vi "CD Storage Library Load.vi"(8 "error in (no error)":errorcluster, 11 "DMA Channel Testing in":refnum<class "FPGA Addon DMA Channel Unit Tests.lvclass">) -> (0 "error out":errorcluster, 3 "DMA Channel Testing out":refnum<class "FPGA Addon DMA Channel Unit Tests.lvclass">)   [LabVIEW 2020, in "FPGA Addon DMA Channel Unit Tests.lvclass"]
uses:
  FPGA Addon DMA Channel Unit Tests.lvclass
  FPGA Addon DMA Channel Unit Tests.lvclass/FPGA Addon DMA Channel Unit Tests.ctl
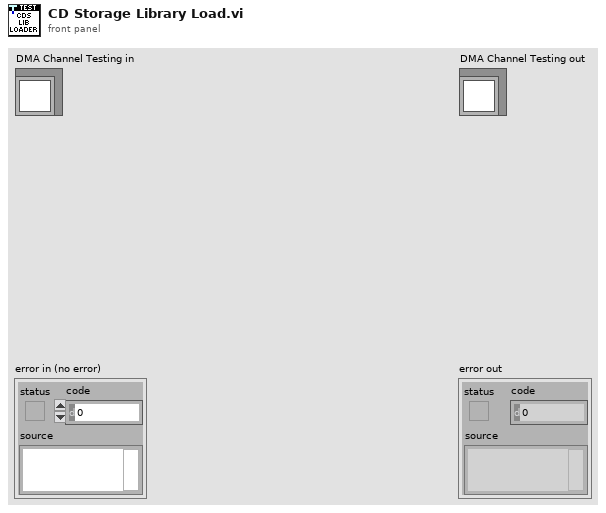
[diagram p1: front panel]
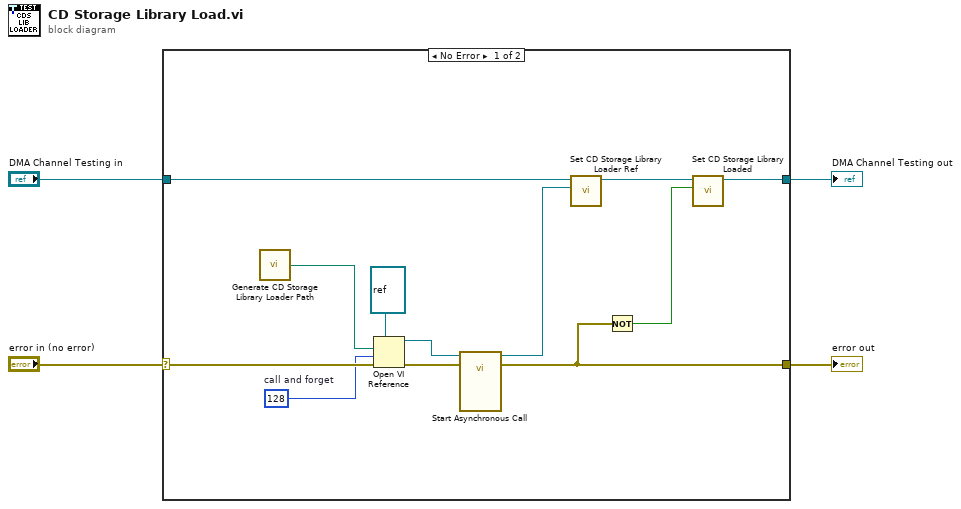
[diagram p0: block diagram]
diagram:
  n1 = case shown="No Error" "error in (no error)" {
    selector: "error in (no error)" -> [w16 w18]
    tunnel: [w15 w18] -> w3
    tunnel: [w10 w17] -> w1
    tunnel: "DMA Channel Testing in" -> [w14 w17]
    frame No Error {
      w8 = 128  # call and forget
      n2 = call "Generate CD Storage Library Loader Path.vi"() -> ("CDS Loader path"=w9:path)
      n3 = Open VI Reference(type specifier VI Refnum (for type only)=refnum<vi> refnum, vi path=w9, options=w8, error in (no error)=w16) -> (vi reference=w5:refnum<vi>, error out=w6:errorcluster)  [unwired: 2 in]
      n4 = call-by-ref "Start Asynchronous Call"(reference=w5, error in=w6) -> (reference out=w13:refnum<vi>, error out=w15:errorcluster)  [unwired: 12 in]
      n5 = call "Set CD Storage Library Loader Ref.vi"("CDS Loader Ref"=w13, "DMA Channel Testing in"=w14) -> ("DMA Channel Testing out"=w12:refnum<class "FPGA Addon DMA Channel Unit Tests.lvclass">)  [unwired: 9 in]
      n6 = Not(x=w15) -> (.not. x?=w11:bool)
      n7 = call "Set CD Storage Library Loaded.vi"("CDS Loaded"=w11, "DMA Channel Testing in"=w12) -> ("DMA Channel Testing out"=w10:refnum<class "FPGA Addon DMA Channel Unit Tests.lvclass">)  [unwired: 9 in]
    }
    frame Error {
    }
  }
  "error out" <- w3
  "DMA Channel Testing out" <- w1
